vi "Func - FuncVI Refnums (Open Ref Type 1).vi"(8 "error in":errorcluster, 9 "options":i32 format="%.0x", 10 "vi path":path) -> (0 "error out":errorcluster, 3 "FuncVI RefNum":refnum<vi>)   [LabVIEW 2021]
doc: "::: CalcExpress Toolkit :::\nCopyright (c) 2000-2026 Konstantin Shifershteyn. All rights reserved."
panel:
  in  "FuncVI RefNum Template":refnum<vi>
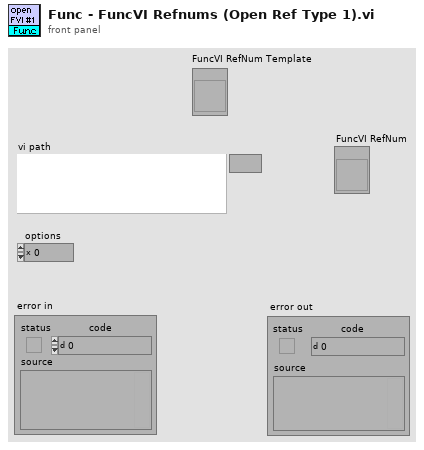
[diagram p1: front panel]
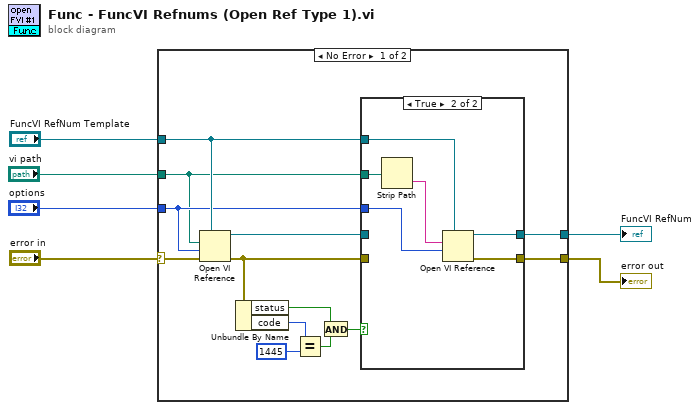
[diagram p0: block diagram]
diagram:
  n1 = case shown="No Error" "error in" {
    selector: "error in" -> [w7 w28]
    tunnel: "FuncVI RefNum Template" -> [w14 _]
    tunnel: "options" -> [w12 _]
    tunnel: "vi path" -> [w11 _]
    tunnel: [w10 _] -> w3
    tunnel: [w9 w28] -> w2
    frame No Error {
      n2 = Open VI Reference(type specifier VI Refnum (for type only)=w14, vi path=w11, options=w12, error in (no error)=w7) -> (vi reference=w15:refnum<vi>, error out=w8:errorcluster)  [unwired: 2 in]
      n3 = Unbundle By Name(w8) -> ("status"=w17:bool, "code"=w19:i32)
      n4 = Equal?(x=w19, y=1445) -> (x = y?=w16:bool)
      n5 = And(x=w17, y=w16) -> (x .and. y?=w13:bool)
      n6 = case shown="True" w13 {
        tunnel: [w21 w26] -> w10
        tunnel: w15 -> [w21 _]
        tunnel: w14 -> [_ w27]
        tunnel: w12 -> [_ w25]
        tunnel: w11 -> [_ w24]
        tunnel: [w20 w22] -> w9
        tunnel: w8 -> [w20 _]
        frame False {
        }
        frame True {
          n7 = Strip Path(path=w24) -> (name=w23:string)  [unwired: 1 out]
          n8 = Open VI Reference(type specifier VI Refnum (for type only)=w27, vi path=w23, options=w25) -> (vi reference=w26:refnum<vi>, error out=w22:errorcluster)  [unwired: 3 in]
        }
      }
    }
    frame Error {
    }
  }
  "error out" <- w2
  "FuncVI RefNum" <- w3
